vi "RemoveChannel.vi"(8 "error in (no error)":errorcluster, 10 "Name":string, 11 "object in":refnum<class "ChannelsManager.lvclass">) -> (0 "error out":errorcluster, 3 "object out":refnum<class "ChannelsManager.lvclass">)   [LabVIEW 2021, in "Channel.lvlib" / "ChannelsManager.lvlib" / "ChannelsManager.lvclass"]
doc: "Adds the channel"
uses:
  ChannelsManager.lvclass
  ChannelsManager.lvclass/ChannelsManager.ctl
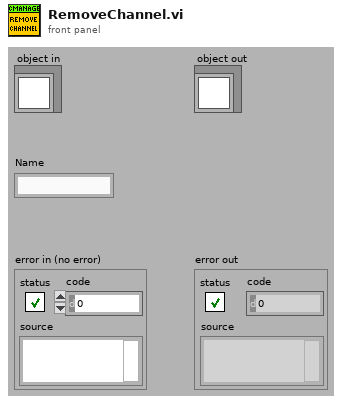
[diagram p1: front panel]
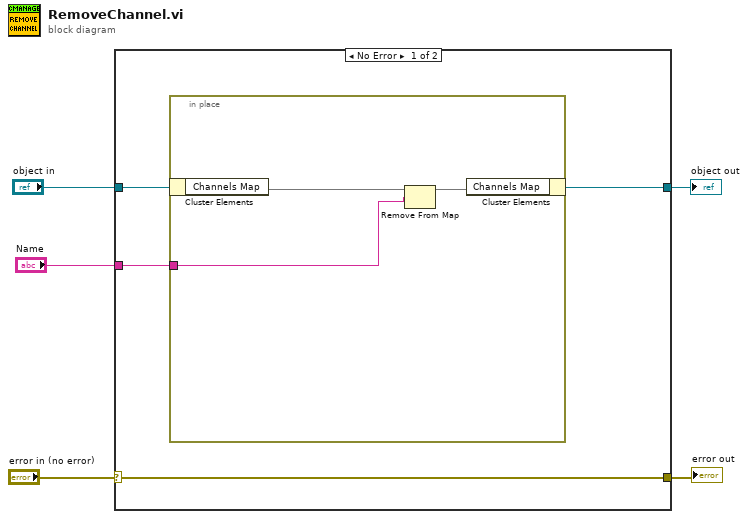
[diagram p0: block diagram]
diagram:
  n1 = case shown="No Error" "error in (no error)" {
    selector: "error in (no error)" -> [w9 w14]
    tunnel: [w9 w14] -> w4
    tunnel: [w7 w13] -> w2
    tunnel: "object in" -> [w8 w13]
    tunnel: "Name" -> [w6 _]
    frame No Error {
      n2 = in-place {
        in-place-border: w6 -> [w10]
        n3 = in-place-cluster #1(w8) -> ("Channels Map"=w12:map{string, refnum<class "Channel.lvclass">})
        n4 = Remove From Map(10:w10, 11:w12) -> (3:w11:map{string, refnum<class "Channel.lvclass">})  [unwired: 2 out]
        n5 = in-place-cluster #1("Channels Map"=w11) -> (w7:refnum<class "ChannelsManager.lvclass">)
      }
    }
    frame Error {
    }
  }
  "error out" <- w4
  "object out" <- w2
